vi "lvmcp_rep.vi"() -> ()   [LabVIEW 2026]
panel:
  out "error out":errorcluster
  in  "representation":u16
  in  "reference":refnum<vi>
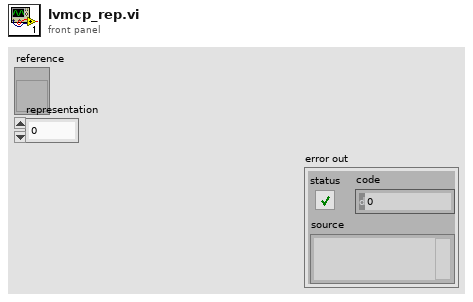
[diagram p1: front panel]
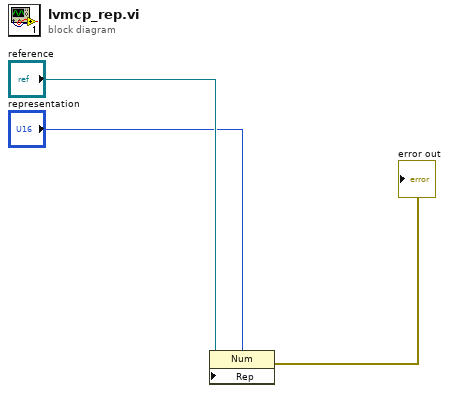
[diagram p0: block diagram]
diagram:
  n1 = property class="Num"(reference="reference", "Rep"="representation") -> (error out=→"error out":errorcluster)  [unwired: 1 in, 1 out]
